vi "ZM-HWM-createEvents.vi"(8 "error in (no error)":errorcluster, 11 "ZM-HWM-hardware_manager in":refnum<class "ZM-HWM-hardware_manager.lvclass">) -> (0 "error out":errorcluster, 3 "ZM-HWM-hardware_manager out":refnum<class "ZM-HWM-hardware_manager.lvclass">)   [LabVIEW 2020, in "ZM-HWM-hardware_manager.lvlib" / "ZM-HWM-hardware_manager.lvclass"]
doc: "Creates the hardware manager's stop user event and stores it in the events field (ZM-HWM-EVENTS). Called by ZM-HWM-createResources; the error goes out so a failed create fails the launch."
uses:
  ZM-HWM-hardware_manager.lvclass
  ZM-HWM-hardware_manager.lvclass/ZM-HWM-hardware_manager.ctl
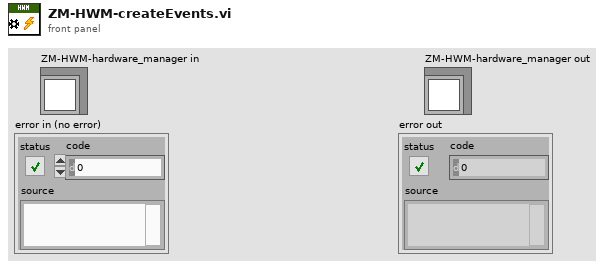
[diagram p1: front panel]
types:
  T1 = typedef "ZM-HWM-hardware_manager.lvlib/ZM-HWM-hardware_manager.lvclass/ZM-HWM-EVENTS.ctl" = cluster{"stop":refnum<user-event>}
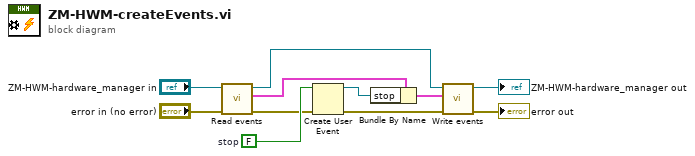
[diagram p0: block diagram]
diagram:
  w9 = FALSE  # stop
  n1 = call "Read events.vi"("error in (no error)"="error in (no error)", "ZM-HWM-hardware_manager in"="ZM-HWM-hardware_manager in") -> ("error out"=w8:errorcluster, "ZM-HWM-EVENTS"=w6:T1, "ZM-HWM-hardware_manager out"=w4:refnum<class "ZM-HWM-hardware_manager.lvclass">)  [unwired: 7 in]
  n2 = Create User Event(user event datatype=w9, error in=w8) -> (user event=w7:refnum<user-event>, error out=w5:errorcluster)
  n3 = Bundle By Name(cluster=w6, "stop"=w7) -> (w3:T1)
  n4 = call "Write events.vi"("error in (no error)"=w5, "ZM-HWM-EVENTS"=w3, "ZM-HWM-hardware_manager in"=w4) -> ("error out"=→"error out":errorcluster, "ZM-HWM-hardware_manager out"=→"ZM-HWM-hardware_manager out":refnum<class "ZM-HWM-hardware_manager.lvclass">)  [unwired: 7 in]
